vi "SaveCFG.vi"(7 "Clear Before Saving(F)":bool, 8 "error in (no error)":errorcluster, 11 "object in":refnum<class "AIO-Configuration.lvclass">) -> (0 "error out":errorcluster, 2 "OK?":bool, 3 "object out":refnum<class "AIO-Configuration.lvclass">)   [LabVIEW 2021, in "DAQmx.lvlib" / "AIO-Configuration.lvclass"]
doc: "Saves Configuration"
uses:
  AIO-Configuration.lvclass
  C:/Users/averna/Documents/LV Gym DEMO/Factory Pattern/Channels/Dependencies/Channel.lvlibp/Channel/Configuration_class/Configuration.lvclass
  Dependencies/Channel.lvlibp/Channel/Configuration_class/properties/ReadConfigurationFile.vi
  <vilib>/Utility/config.llb/Write Key (String).vi
  <vilib>/Utility/config.llb/Write Key (Double).vi
  Dependencies/AIO-Channel.lvlibp/AIO-Configuration_class/AIO-Configuration.lvclass
  <vilib>/Utility/config.llb/NI_LVConfig.lvlib
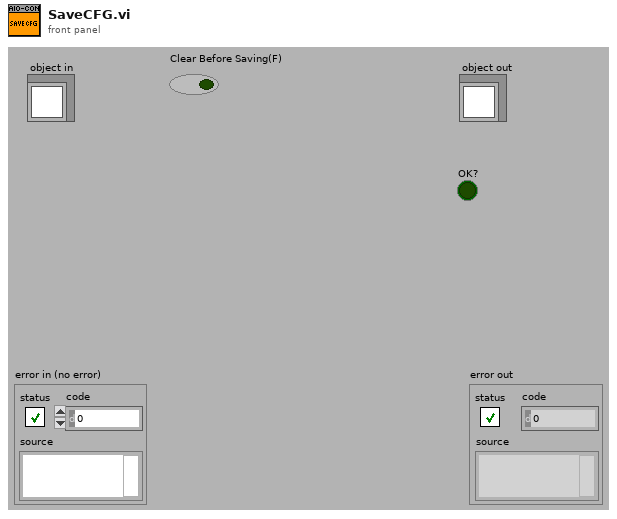
[diagram p1: front panel]
types:
  T1 = typedef "NI_LVConfig.lvlib/Config Data RefNum.ctl" = refnum<k1>
  T2 = typedef "DAQmx.lvlib/AIO-Configuration.lvclass/Data.ctl" = cluster{"DAQ_Line":string, "maximum value":dbl, "minimum value":dbl, "input terminal configuration":i32, "custom scale name":string}
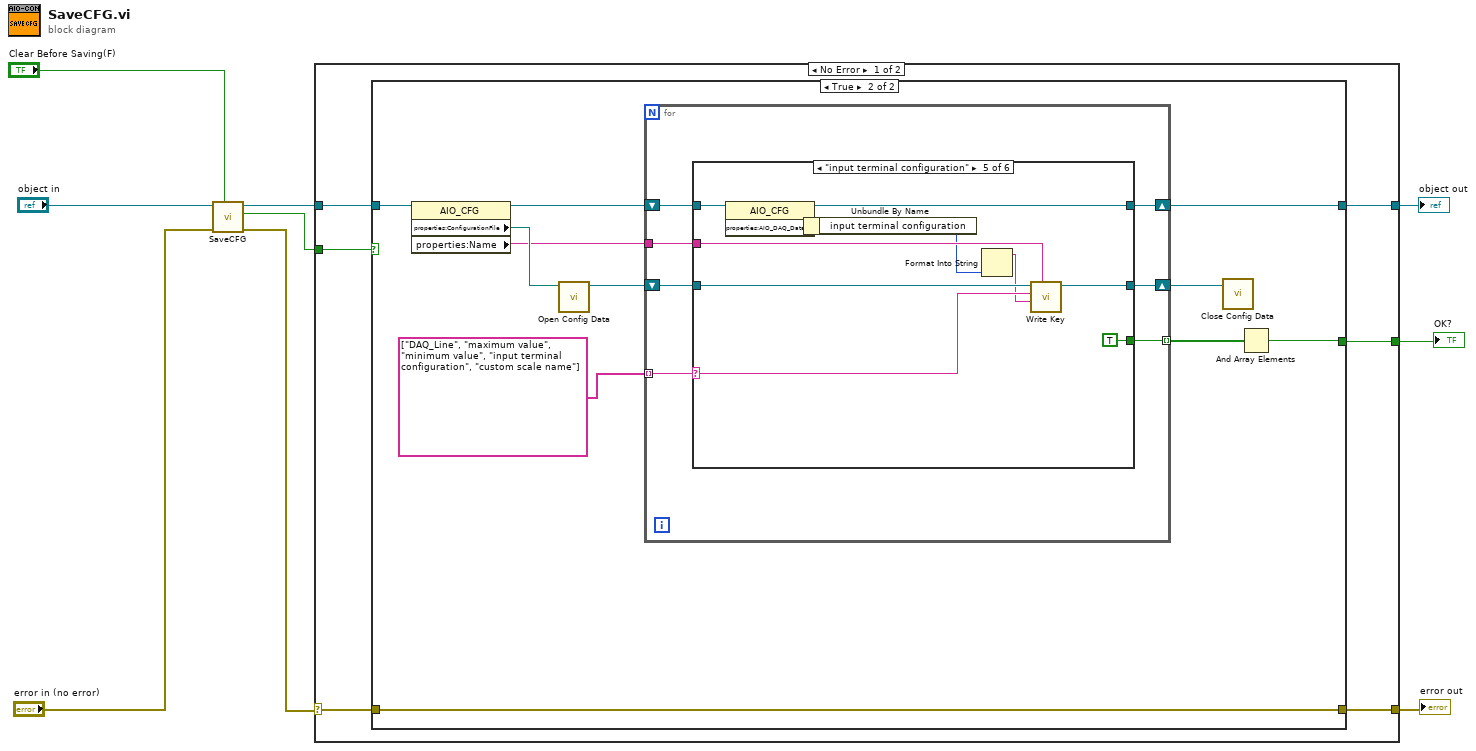
[diagram p0: block diagram]
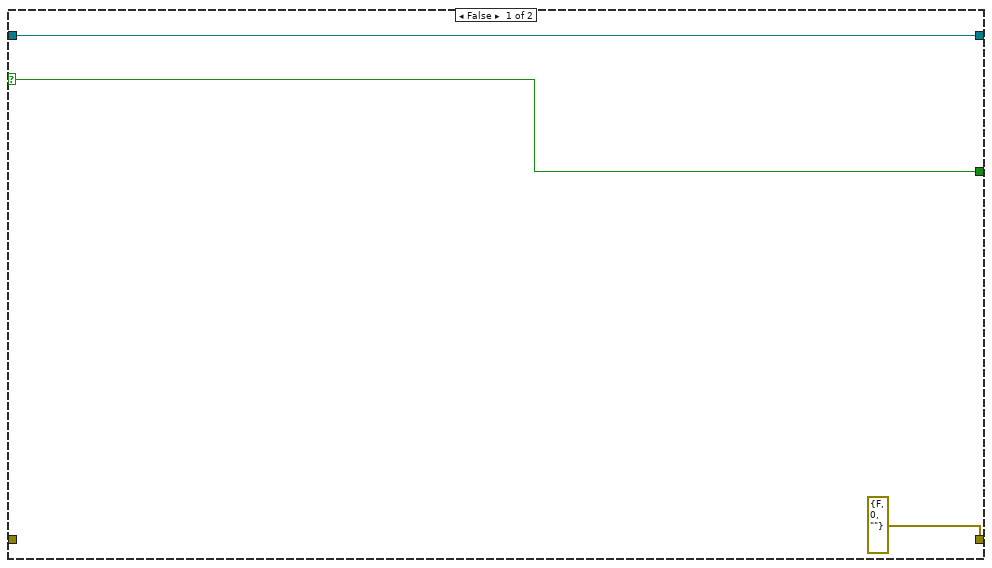
[diagram p2: hidden frame]
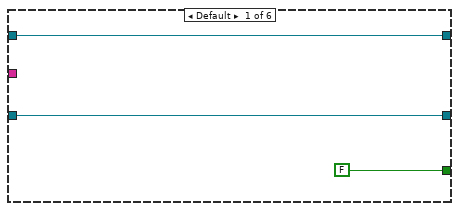
[diagram p3: hidden frame]
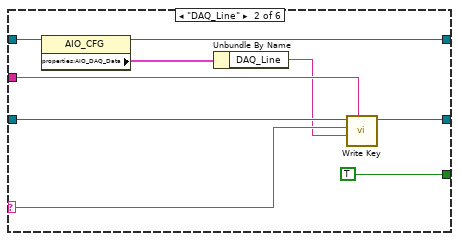
[diagram p4: hidden frame]
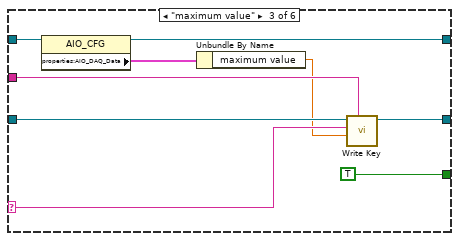
[diagram p5: hidden frame]
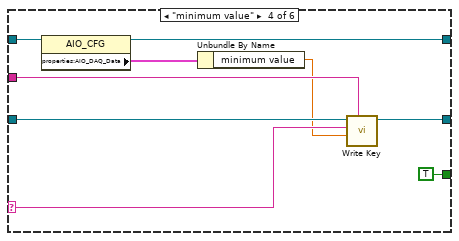
[diagram p6: hidden frame]
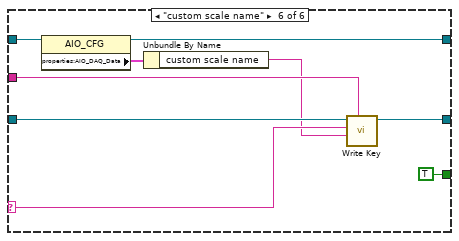
[diagram p7: hidden frame]
diagram:
  n1 = call-parent "SaveCFG.vi"("Clear Before Saving(F)"="Clear Before Saving(F)", "error in (no error)"="error in (no error)", "object in"="object in") -> ("error out"=w5:errorcluster, "OK?"=w3:bool, "object out"=w7:refnum<class "AIO-Configuration.lvclass">)  [unwired: 6 in]
  n2 = case shown="No Error" w5 {
    selector: w5 -> [w12 w88]
    tunnel: [w13 w88] -> w9
    tunnel: w7 -> [w14 w87]
    tunnel: [w10 w86] -> w2
    tunnel: w3 -> [w11 w86]
    tunnel: [w15 w87] -> w1
    frame No Error {
      n3 = case shown="True" w11 {
        selector: w11 -> [w17 _]
        tunnel: [w18 w25] -> w15
        tunnel: w14 -> [w18 w29]
        tunnel: [errorcluster {"status"=FALSE, "code"=0, "source"=""} ("error IO") w28] -> w13
        tunnel: w12 -> [_ w28]
        tunnel: [w17 w20] -> w10
        frame False {
        }
        frame True {
          n4 = property class="AIO_CFG"(reference=w29) -> (reference out=w24:refnum<class "AIO-Configuration.lvclass">, "properties:ConfigurationFile"=w27:path, "properties:Name"=w22:string)  [unwired: 1 in, 1 out]
          n5 = call <vilib>:"Open Config Data.vi"("configuration file path"=w27) -> ("refnum"=w26:T1)  [unwired: 8 in, 2 out]
          n6 = for {
            shift-right: [w32] -> w25
            shift-left: w24 -> [w31]
            shift-right: [w35] -> w23
            shift-left: w26 -> [w36]
            tunnel: string[] ["DAQ_Line", "maximum value", "minimum value", "input terminal configuration", "custom scale name"] -> [w34] mode=indexing
            tunnel: w22 -> [w33]
            tunnel: [w30] -> w21 mode=indexing
            n7 = case shown="\"input terminal configuration\"" w34 {
              selector: w34 -> [_ w46 w55 w64 w74 w83]
              tunnel: w36 -> [w38 w48 w57 w66 w76 w85]
              tunnel: [w38 w47 w56 w65 w75 w84] -> w35
              tunnel: w33 -> [_ w45 w54 w63 w73 w82]
              tunnel: [w39 w43 w52 w61 w71 w80] -> w32
              tunnel: w31 -> [w39 w44 w53 w62 w72 w81]
              tunnel: [FALSE ("found?") TRUE ("found?") TRUE ("found?") TRUE ("found?") TRUE ("found?") TRUE ("found?")] -> w30
              frame Default {
              }
              frame "DAQ_Line" {
                n8 = property class="AIO_CFG"(reference=w44) -> (reference out=w43:refnum<class "AIO-Configuration.lvclass">, "properties:AIO_DAQ_Data"=w42:T2)  [unwired: 1 in, 1 out]
                n9 = Unbundle By Name(w42) -> ("DAQ_Line"=w41:string)
                n10 = call-poly <vilib>:"Write Key.vi"("section"=w45, "value"=w41, "key"=w46, "refnum"=w48) -> ("refnum out"=w47:T1)  [unwired: 5 in, 2 out]
              }
              frame "maximum value" {
                n11 = property class="AIO_CFG"(reference=w53) -> (reference out=w52:refnum<class "AIO-Configuration.lvclass">, "properties:AIO_DAQ_Data"=w51:T2)  [unwired: 1 in, 1 out]
                n12 = Unbundle By Name(w51) -> ("maximum value"=w50:dbl)
                n13 = call-poly <vilib>:"Write Key.vi"("section"=w54, "value"=w50, "key"=w55, "refnum"=w57) -> ("refnum out"=w56:T1)  [unwired: 5 in, 2 out]
              }
              frame "minimum value" {
                n14 = property class="AIO_CFG"(reference=w62) -> (reference out=w61:refnum<class "AIO-Configuration.lvclass">, "properties:AIO_DAQ_Data"=w60:T2)  [unwired: 1 in, 1 out]
                n15 = Unbundle By Name(w60) -> ("minimum value"=w59:dbl)
                n16 = call-poly <vilib>:"Write Key.vi"("section"=w63, "value"=w59, "key"=w64, "refnum"=w66) -> ("refnum out"=w65:T1)  [unwired: 5 in, 2 out]
              }
              frame "input terminal configuration" {
                n17 = property class="AIO_CFG"(reference=w72) -> (reference out=w71:refnum<class "AIO-Configuration.lvclass">, "properties:AIO_DAQ_Data"=w70:T2)  [unwired: 1 in, 1 out]
                n18 = Unbundle By Name(w70) -> ("input terminal configuration"=w68:i32)
                n19 = Format Into String(w68) -> (resulting string=w67:string)  [unwired: 3 in, 1 out]
                n20 = call-poly <vilib>:"Write Key.vi"("section"=w73, "value"=w67, "key"=w74, "refnum"=w76) -> ("refnum out"=w75:T1)  [unwired: 5 in, 2 out]
              }
              frame "custom scale name" {
                n21 = property class="AIO_CFG"(reference=w81) -> (reference out=w80:refnum<class "AIO-Configuration.lvclass">, "properties:AIO_DAQ_Data"=w79:T2)  [unwired: 1 in, 1 out]
                n22 = Unbundle By Name(w79) -> ("custom scale name"=w77:string)
                n23 = call-poly <vilib>:"Write Key.vi"("section"=w82, "value"=w77, "key"=w83, "refnum"=w85) -> ("refnum out"=w84:T1)  [unwired: 5 in, 2 out]
              }
            }
          }
          n24 = call <vilib>:"Close Config Data.vi"("refnum"=w23) -> ()  [unwired: 9 in, 2 out]
          n25 = And Array Elements(Boolean array=w21) -> (logical AND=w20:bool)
        }
      }
    }
    frame Error {
    }
  }
  "error out" <- w9
  "object out" <- w1
  "OK?" <- w2
